vi "ZM-PC-TP-setType.vi"(8 "error in (no error)":errorcluster, 11 "ZM-PC-package in":refnum<class "ZM-PC-package.lvclass">) -> (0 "error out":errorcluster, 3 "ZM-PC-package out":refnum<class "ZM-PC-package.lvclass">)   [LabVIEW 2020, in "ZM-PC-packages.lvlib" / "ZM-PC-TP-test_package.lvclass"]
doc: "Hook of the test package: writes the type TestPackage through the parent's Write type. Both class terminals are typed ZM-PC-package so that the hook sits between Call Parent and the dynamic output of the init override (a static VI with the same class in and out keeps the run-time type)."
uses:
  ZM-PC-TP-test_package.lvclass
  ZM-PC-package/ZM-PC-package.lvclass
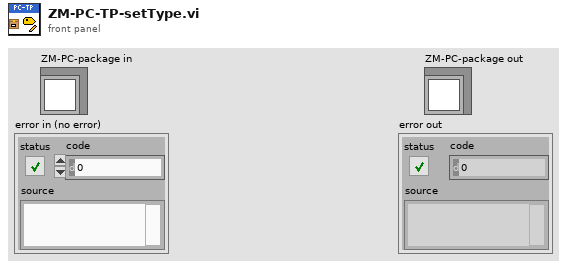
[diagram p1: front panel]
types:
  T1 = enum16{"Undefined", "TestPackage", "ErrorPackage"}
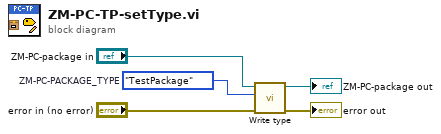
[diagram p0: block diagram]
diagram:
  w3 = T1."TestPackage"  # ZM-PC-PACKAGE_TYPE
  n1 = call "Write type.vi"("error in (no error)"="error in (no error)", "ZM-PC-PACKAGE_TYPE"=w3, "ZM-PC-package in"="ZM-PC-package in") -> ("error out"=→"error out":errorcluster, "ZM-PC-package out"=→"ZM-PC-package out":refnum<class "ZM-PC-package.lvclass">)  [unwired: 7 in]
